vi "Test round to nearest.vi"() -> ()   [LabVIEW 2019]
panel:
  in  "Round to nearest":dbl=11.0
  in  "BP":dbl
  out "New BP":dbl
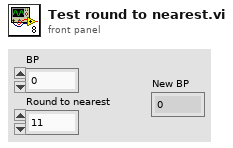
[diagram p1: front panel]
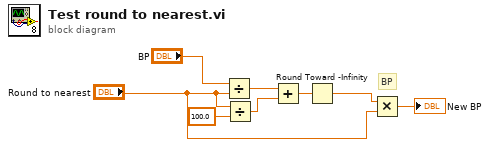
[diagram p0: block diagram]
diagram:
  # "BP"
  n1 = Divide(x="BP", y="Round to nearest") -> (x/y=w8:dbl)
  n2 = Divide(x="Round to nearest", y=100.0) -> (x/y=w5:dbl)
  n3 = Add(x=w8, y=w5) -> (x+y=w7:dbl)
  n4 = Round Toward -Infinity(1:w7) -> (0:w6:dbl)
  n5 = Multiply(x=w6, y="Round to nearest") -> (x*y=→"New BP":dbl)
